vi "Decor.Numeric.vi"(7 "VI ref":refnum<vi>, 8 "error in (no error)":errorcluster, 10 "ctrl ref in":refnum<vi>, 11 "Material-Scheme in":refnum<class "Material-Scheme.lvclass">) -> (0 "error out":errorcluster)   [LabVIEW 2021, in "TSC Material Theme.lvlib" / "Material-Scheme.lvclass"]
uses:
  Material-Scheme.lvclass
  Material-Scheme.lvclass/Material-Scheme.ctl
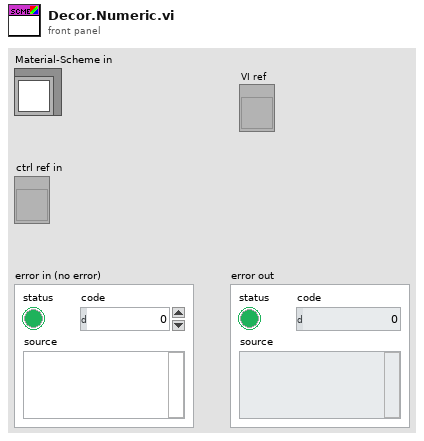
[diagram p1: front panel]
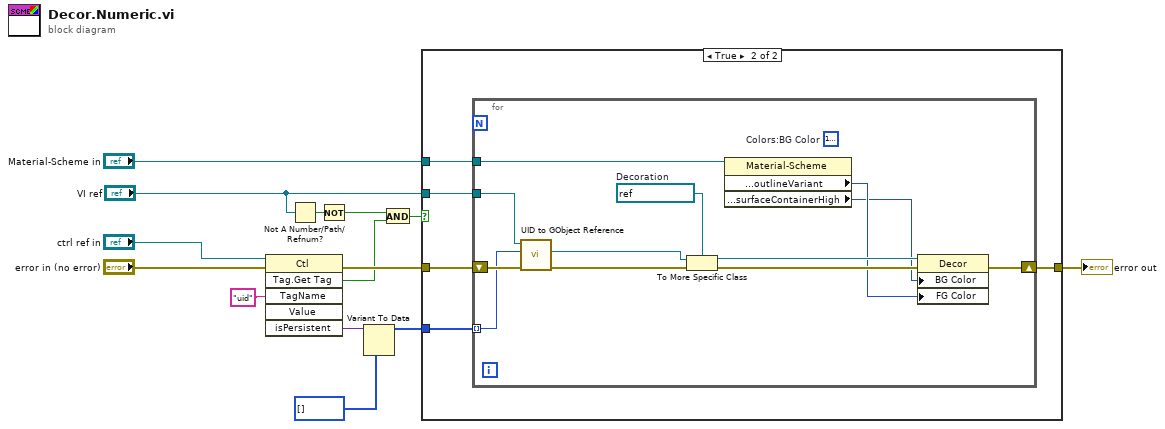
[diagram p0: block diagram]
diagram:
  n1 = invoke class="Ctl" method="Tag.Get Tag"(reference="ctrl ref in", error in="error in (no error)", "TagName"="uid" ("Tag Name")) -> (error out=w9:errorcluster, "GetTag"=w5:bool, "isPersistent"=w13:variant)  [unwired: 3 in, 3 out]
  n2 = Not A Number/Path/Refnum?(number/path/refnum="VI ref") -> (NaN/Path/Refnum?=w3:bool)
  n3 = Not(x=w3) -> (.not. x?=w2:bool)
  n4 = Variant To Data(type=i32[] [], Variant=w13) -> (data=w7:i32[])  [unwired: 1 in, 1 out]
  n5 = And(x=w2, y=w5) -> (x .and. y?=w1:bool)
  n6 = case shown="True" w1 {
    tunnel: w9 -> [w15 w20]
    tunnel: [w15 w19] -> w8
    tunnel: "VI ref" -> [_ w18]
    tunnel: w7 -> [_ w17]
    tunnel: "Material-Scheme in" -> [_ w16]
    frame False {
    }
    frame True {
      n7 = for {
        tunnel: w18 -> [w30]
        shift-right: [w25] -> w19
        shift-left: w20 -> [w32]
        tunnel: w17 -> [w29] mode=indexing
        tunnel: w16 -> [w23]
        (unwired) u32 16777216  # Colors:BG Color
        w26 = refnum<vi> refnum  # Decoration
        n8 = call <vilib>:"UID to GObject Reference.vi"("error in (no error)"=w32, "UID"=w29, "Owning VI"=w30) -> ("error out"=w31:errorcluster, "GObject"=w27:refnum<vi>)  [unwired: 6 in, 1 out]
        n9 = To More Specific Class(target class=w26, reference=w27, error in=w31) -> (specific class reference=w24:refnum<vi>, error out=w28:errorcluster)
        n10 = property class="Material-Scheme"(reference=w23) -> ("data member access:Other:outlineVariant"=w22:u32, "data member access:Surface:surfaceContainerHigh"=w21:u32)  [unwired: 1 in, 2 out]
        n11 = property class="Decor"(reference=w24, error in=w28, "BG Color"=w21, "FG Color"=w22) -> (error out=w25:errorcluster)  [unwired: 1 out]
      }
    }
  }
  "error out" <- w8
